vi "check Event Status Bit for OPC.vi"(8 "error in (no error)":errorcluster, 11 "Keysight 9020A in":refnum<class "Keysight 9020A.lvclass">) -> (0 "error out":errorcluster, 2 "OPC Bit Changed?":bool, 3 "Keysight 9020A out":refnum<class "Keysight 9020A.lvclass">)   [LabVIEW 2023, in "Spectrum Analyzer.lvlib" / "Keysight 9020A.lvclass"]
uses:
  Keysight 9020A.lvclass
  Keysight 9020A.lvclass/Keysight 9020A.ctl
  Spectrum Analyzer.lvlib
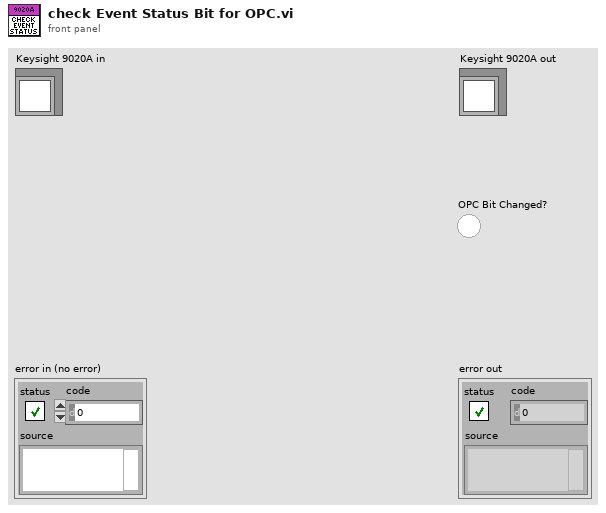
[diagram p1: front panel]
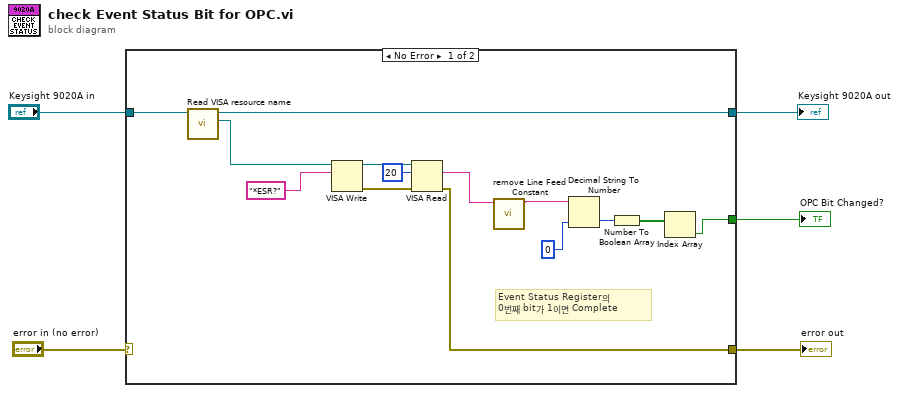
[diagram p0: block diagram]
diagram:
  n1 = case shown="No Error" "error in (no error)" {
    selector: "error in (no error)" -> [_ w20]
    tunnel: "Keysight 9020A in" -> [w19 w21]
    tunnel: [w18 w21] -> w3
    tunnel: [w6 w20] -> w2
    tunnel: [w7 _] -> w1
    frame No Error {
      # "Event Status Register의\n0번째 bit가 1이면 Complete"
      n2 = call "Read VISA resource name.vi"("Keysight 9020A in"=w19) -> ("VISA resource name"=w13:refnum<visa-resource-name>, "Keysight 9020A out"=w18:refnum<class "Keysight 9020A.lvclass">)  [unwired: 8 in, 1 out]
      n3 = VISA Write(VISA resource name=w13, write buffer="*ESR?") -> (VISA resource name out=w16:refnum<visa-resource-name>, error out=w15:errorcluster)  [unwired: 1 in, 1 out]
      n4 = VISA Read(VISA resource name=w16, byte count=u32 20, error in (no error)=w15) -> (read buffer=w12:string, error out=w6:errorcluster)  [unwired: 2 out]
      n5 = call "remove Line Feed Constant.vi"("Input String"=w12) -> ("Line Feed Removed String"=w9:string)  [unwired: 10 in]
      n6 = Decimal String To Number(string=w9, default (0L)=i16 0) -> (number=w10:i16)  [unwired: 1 in, 1 out]
      n7 = Number To Boolean Array(number=w10) -> (Boolean array=w8:bool[])
      n8 = Index Array(array=w8) -> (element=w7:bool)  [unwired: 1 in]
    }
    frame Error {
    }
  }
  "error out" <- w2
  "Keysight 9020A out" <- w3
  "OPC Bit Changed?" <- w1
